vi "Connect.vi"(8 "error in (no error)":errorcluster, 11 "object in":refnum<class "Channel.lvclass">) -> (0 "error out":errorcluster, 2 "Success?":bool, 3 "object out":refnum<class "Channel.lvclass">)   [LabVIEW 2021, in "Channel.lvlib" / "Channel.lvclass"]
doc: "Connects the channel using the current Configuration"
uses:
  Channel.lvclass
  Channel.lvclass/Channel.ctl
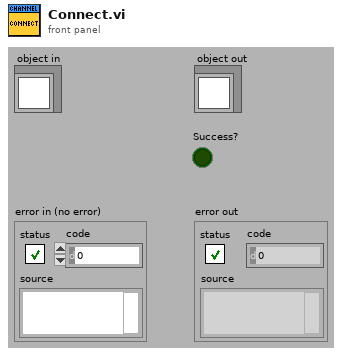
[diagram p1: front panel]
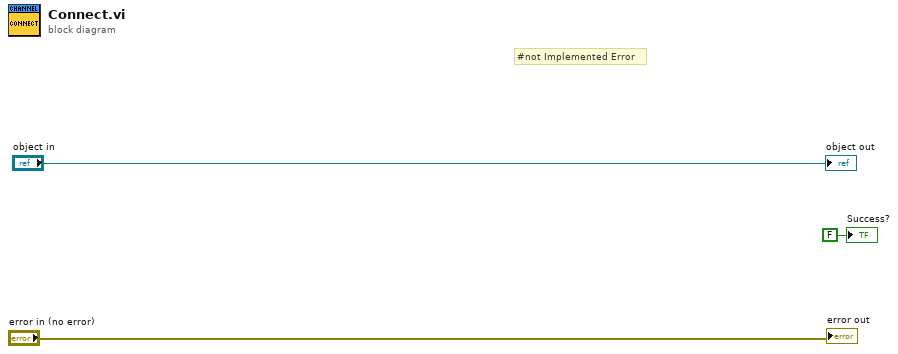
[diagram p0: block diagram]
diagram:
  # "#not Implemented Error"
  "error out" <- "error in (no error)"
  "object out" <- "object in"
  "Success?" <- FALSE ("Success?")
